vi "Read String Inputs.vi"(8 "error in (no error)":errorcluster, 11 "Modbus in":refnum<class "Modbus.lvclass">) -> (0 "error out":errorcluster, 3 "Modbus out":refnum<class "Modbus.lvclass">)   [LabVIEW 2026, in "Modbus.lvlib" / "Modbus.lvclass"]
uses:
  Modbus.lvclass
  C:/Program Files/National Instruments/LabVIEW 2026/vi.lib/FlexLogger/SDK/PluginSDK.lvlibp/PEFClasses/SDK/Plugin/Plugin.lvclass
  Modbus.lvclass/Modbus.ctl
  <vilib>/FlexLogger/SDK/PluginSDK.lvlibp/PEFClasses/SDK/Plugin/DataHelpers/Write 1D STR (NChan 1 Sample).vi
  C:/Program Files/National Instruments/LabVIEW 2026/vi.lib/FlexLogger/SDK/PluginSDK.lvlibp/PEFClasses/SDK/Processing Element/Processing Element.lvclass
  D:/Work/FlexLogger/Features/Modbus Plugin/Modbus - Working Copy/Modbus/Modbus.lvclass
  <vilib>/FlexLogger/SDK/PluginSDK.lvlibp/PEFClasses/SDK/Plugin/Plugin.lvclass
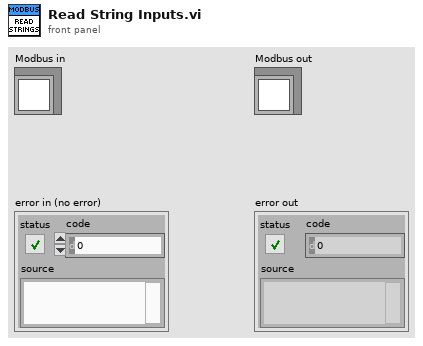
[diagram p1: front panel]
types:
  T1 = typedef "Modbus.lvlib/Modbus.lvclass/String Data.ctl" = cluster{"Channel UID":string, "Valid?":bool, "Table":T2, "Address":i32, "Quantity":u16}
  T2 = typedef "Modbus.lvlib/Modbus.lvclass/Modbus Table.ctl" = enum16{"Discrete Inputs", "Coils", "Input Registers", "Holding Registers"}
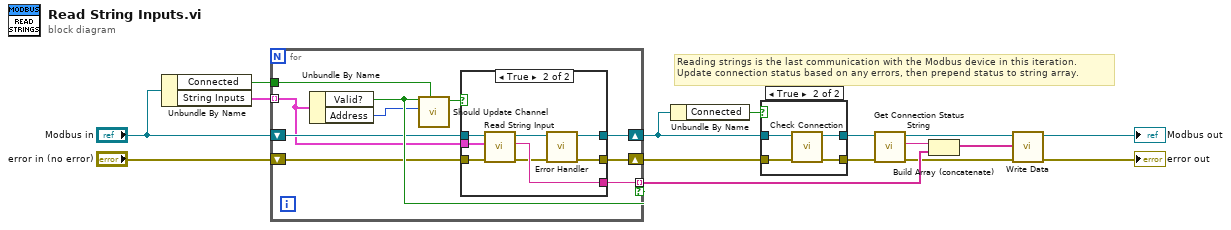
[diagram p0: block diagram]
diagram:
  # "Reading strings is the last communication with the Modbus device in this iteration.\nUpdate connection status based on any errors, then prepend status to string array."
  n1 = Unbundle By Name("Modbus in") -> ("Connected"=w14:bool, "String Inputs"=w1:T1[])
  n2 = for {
    tunnel: w1 -> [w18] mode=indexing
    tunnel: [w26] -> w12 mode=indexing if=w25
    shift-right: [w22] -> w8
    shift-left: "error in (no error)" -> [w23]
    tunnel: w14 -> [w21]
    shift-right: [w19] -> w9
    shift-left: "Modbus in" -> [w20]
    n3 = Unbundle By Name(w18) -> ("Valid?"=w25:bool, "Address"=w17:i32)
    n4 = call "Should Update Channel.vi"("Connected?"=w21, "Address"=w17, "Valid?"=w25) -> ("Update?"=w24:bool)  [unwired: 8 in]
    n5 = case shown="True" w24 {
      tunnel: [w28 w35] -> w22
      tunnel: [_ w31] -> w26
      tunnel: w23 -> [w28 w36]
      tunnel: w20 -> [w27 w33]
      tunnel: [w27 w34] -> w19
      tunnel: w18 -> [_ w32]
      frame False {
      }
      frame True {
        n6 = call "Read String Input.vi"("error in (no error)"=w36, "String Input in"=w32, "Modbus in"=w33) -> ("error out"=w29:errorcluster, "String Value"=w31:string, "Modbus out"=w30:refnum<class "Modbus.lvclass">)  [unwired: 6 in]
        n7 = call "Error Handler.vi"("error in (no error)"=w29, "Modbus in"=w30) -> ("error out"=w35:errorcluster, "Modbus out"=w34:refnum<class "Modbus.lvclass">)  [unwired: 8 in]
      }
    }
  }
  n8 = Unbundle By Name(w9) -> ("Connected"=w10:bool)
  n9 = case shown="True" w10 {
    tunnel: w8 -> [w37 w42]
    tunnel: [w37 w41] -> w7
    tunnel: w9 -> [w38 w40]
    tunnel: [w38 w39] -> w6
    frame False {
    }
    frame True {
      n10 = call "Check Connection.vi"("error in (no error)"=w42, "Plugin in"=w40) -> ("error out"=w41:errorcluster, "Plugin out"=w39:refnum<class "Modbus.lvclass">)  [unwired: 8 in]
    }
  }
  n11 = call "Get Connection Status String.vi"("error in (no error)"=w7, "Modbus in"=w6) -> ("error out"=w4:errorcluster, "Status String"=w13:string, "Modbus out"=w5:refnum<class "Modbus.lvclass">)  [unwired: 7 in]
  n12 = Build Array (concatenate)(w13, w12) -> (w11:string[])
  n13 = call-poly <vilib>:"Write Data.vi"("error in (no error)"=w4, "Data"=w11, "Plugin in"=w5) -> ("error out"=→"error out":errorcluster, "Plugin out"=→"Modbus out":refnum<class "Modbus.lvclass">)  [unwired: 7 in]
